vi "Read from Hardware.vi"(8 "error in (no error)":errorcluster, 10 "Values in":dbl[](array[numeric]), 11 "Logging Execution Unit in":refnum<class "Logging Execution Unit.lvclass">) -> (0 "error out":errorcluster, 2 "Values out":dbl[](array[numeric]), 3 "Logging Execution Unit out":refnum<class "Logging Execution Unit.lvclass">)   [LabVIEW 2020, in "AIM ARINC 429 Engine.lvlib" / "Implementation.lvlib" / "Logging Execution Unit.lvclass"]
uses:
  Logging Execution Unit.lvclass
  Logging/Word Logging/Word Logging.lvlib
  Execution Unit/Execution Unit.lvclass
  C:/Users/nitest/Desktop/Git 2020/niveristand-aim-arinc429-custom-device/Source/Custom Device Support/Engine/Implementation/Execution Unit/Execution Unit.lvclass
  Hardware API/AIM ARINC 429 Hardware API.lvlib
  Custom Device/Custom Device.lvlib
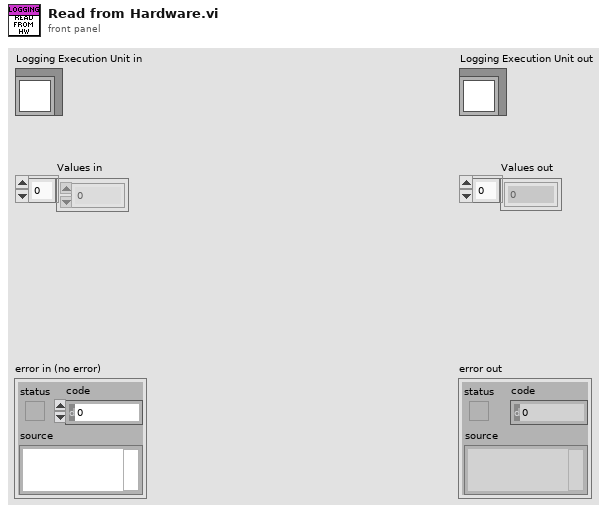
[diagram p1: front panel]
types:
  T1 = typedef "AIM ARINC 429 Hardware API.lvlib/Monitor Data.ctl" = cluster{"time stamp":timestamp, "channel number in":u8, "label":u8, "sdi":u8, "data word":u32}
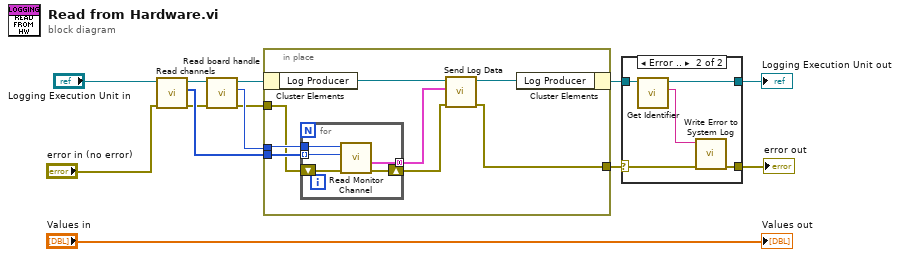
[diagram p0: block diagram]
diagram:
  n1 = call "Read channels.vi"("error in (no error)"="error in (no error)", "Execution Unit in"="Logging Execution Unit in") -> ("error out"=w6:errorcluster, "channels"=w11:u8[], "Execution Unit out"=w10:refnum<class "Logging Execution Unit.lvclass">)  [unwired: 7 in]
  n2 = call "Read board handle.vi"("error in (no error)"=w6, "Execution Unit in"=w10) -> ("error out"=w5:errorcluster, "board handle"=w12:u8, "Execution Unit out"=w9:refnum<class "Logging Execution Unit.lvclass">)  [unwired: 7 in]
  n3 = in-place {
    in-place-border: w12 -> [w19]
    in-place-border: w11 -> [w18]
    in-place-border: w5 -> [w17]
    in-place-border: [w15] -> w2
    n4 = in-place-cluster #1(w9) -> ("Log Producer"=w21:refnum<class "Log Producer.lvclass">)
    n5 = for {
      tunnel: [w22] -> w14 mode=concatenating
      tunnel: w19 -> [w26]
      tunnel: w18 -> [w25] mode=indexing
      shift-right: [w23] -> w16
      shift-left: w17 -> [w24]
      n6 = call "Read Monitor Channel.vi"("error in"=w24, "channel number in"=w25, "board handle in"=w26) -> ("error out"=w23:errorcluster, "monitor data out"=w22:T1[])  [unwired: 5 in, 2 out]
    }
    n7 = call "Send Log Data.vi"("error in (no error)"=w16, "Data"=w14, "Producer in"=w21) -> ("error out"=w15:errorcluster, "Producer out"=w20:refnum<class "Log Producer.lvclass">)  [unwired: 7 in]
    n8 = in-place-cluster #1("Log Producer"=w20) -> (w4:refnum<class "Logging Execution Unit.lvclass">)
  }
  n9 = case shown="Error .." w2 {
    selector: w2 -> [w27 w30]
    tunnel: w4 -> [w28 w33]
    tunnel: [w28 w32] -> w3
    tunnel: [w27 w29] -> w1
    frame No Error {
    }
    frame Error {
      n10 = call-dynamic "Get Identifier.vi"("Execution Unit Implementation in"=w33) -> ("Identifier"=w31:string, "Execution Unit Implementation out"=w32:refnum<class "Logging Execution Unit.lvclass">)  [unwired: 8 in, 1 out]
      n11 = call "Write Error to System Log.vi"("error in"=w30, "identifier"=w31) -> ("error out"=w29:errorcluster)  [unwired: 9 in]
    }
  }
  "error out" <- w1
  "Logging Execution Unit out" <- w3
  "Values out" <- "Values in"
